vi "Disconnect.vi"(8 "error in (no error)":errorcluster, 11 "object in":refnum<class "AIO_Channel.lvclass">) -> (0 "error out":errorcluster, 3 "object out":refnum<class "AIO_Channel.lvclass">)   [LabVIEW 2021, in "Simulator-Channel.lvlib" / "AIO_Channel.lvclass"]
uses:
  AIO_Channel.lvclass
  C:/Users/averna/Documents/LV Gym DEMO/Factory Pattern/Device Channels/Dependencies/AIO-Channel.lvlibp/Channels/AIO-Channel/AIO_Channel_class/AIO_Channel.lvclass
  <vilib>/ActorFramework/Message Enqueuer/Message Enqueuer.lvclass
  AIO_Channel.lvclass/AIO_Channel.ctl
  AIO_Panel/DIO_Panel Messages/Remove Channel Msg/Remove Channel Msg.lvclass/Remove Channel Msg.ctl
  <vilib>/ActorFramework/Message Enqueuer/Message Enqueuer.lvclass/Message Enqueuer.ctl
  <vilib>/ActorFramework/Message Enqueuer/Enqueue.vi
  AIO_Panel/DIO_Panel Messages/Remove Channel Msg/Remove Channel Msg.lvclass
  C:/Program Files/National Instruments/LabVIEW 2021/vi.lib/ActorFramework/Message/Message.lvclass
  Dependencies/AIO-Channel.lvlibp/Channels/AIO-Channel/AIO_Channel_class/Properties/GetAIOConfiguration.vi
  <vilib>/ActorFramework/Message Priority Queue/Priority Enqueue.vi
  Dependencies/AIO-Channel.lvlibp/Channels/AIO-Channel/AIO-Configuration_class/AIO-Configuration.lvclass
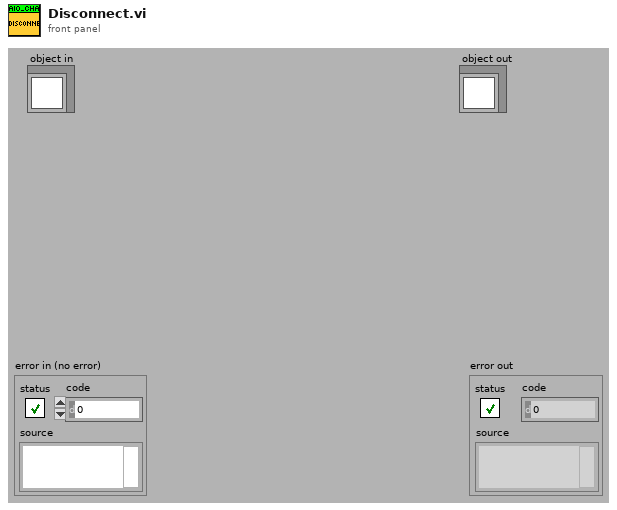
[diagram p1: front panel]
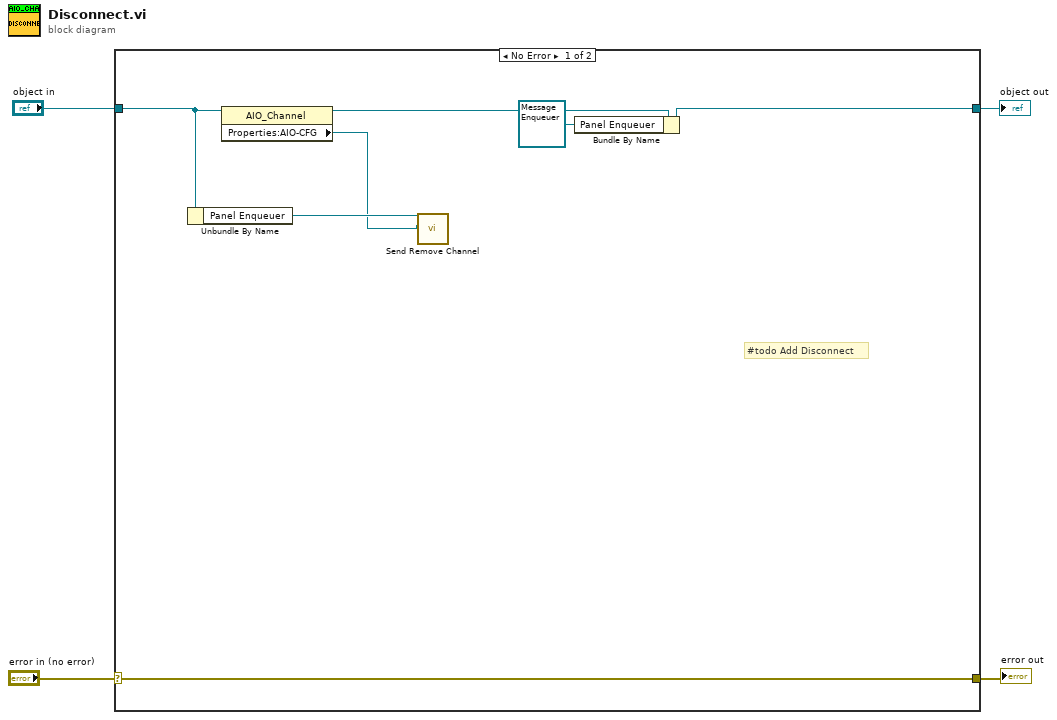
[diagram p0: block diagram]
diagram:
  n1 = case shown="No Error" "error in (no error)" {
    selector: "error in (no error)" -> [w11 w13]
    tunnel: [w11 w13] -> w3
    tunnel: [w9 w12] -> w1
    tunnel: "object in" -> [w10 w12]
    frame No Error {
      # "#todo Add Disconnect"
      n2 = Unbundle By Name(w10) -> ("Panel Enqueuer"=w7:refnum<class "Message Enqueuer.lvclass">)
      n3 = property class="AIO_Channel"(reference=w10) -> (reference out=w6:refnum<class "AIO_Channel.lvclass">, "Properties:AIO-CFG"=w5:refnum<class "AIO-Configuration.lvclass">)  [unwired: 1 in, 1 out]
      n4 = call "Send Remove Channel.vi"("AIO_CFG"=w5, "Message Enqueuer"=w7) -> ()  [unwired: 8 in, 2 out]
      n5 = Bundle By Name(cluster=w6, "Panel Enqueuer"=refnum<class "Message Enqueuer.lvclass"> refnum) -> (w9:refnum<class "AIO_Channel.lvclass">)
    }
    frame Error {
    }
  }
  "error out" <- w3
  "object out" <- w1
